vi "Test - Add Property to Schema.vi"   [LabVIEW 2020, in "JSON Schema Generator.lvlib"]
uses:
  JSON Schema Generator.lvlib
  <vilib>/addons/_JKI Toolkits/Caraya/classes/Test/Test.lvclass
  <vilib>/addons/_JKI Toolkits/Caraya/classes/Assert/Assert.lvclass
  <vilib>/JDP Science/JSONtext/JSONtext.lvlib
  <vilib>/addons/_JKI Toolkits/Caraya/classes/Assert/Assert Equal Value_Variant.vi
  <vilib>/addons/_JKI Toolkits/Caraya/classes/Assert/Assert Not Error.vi
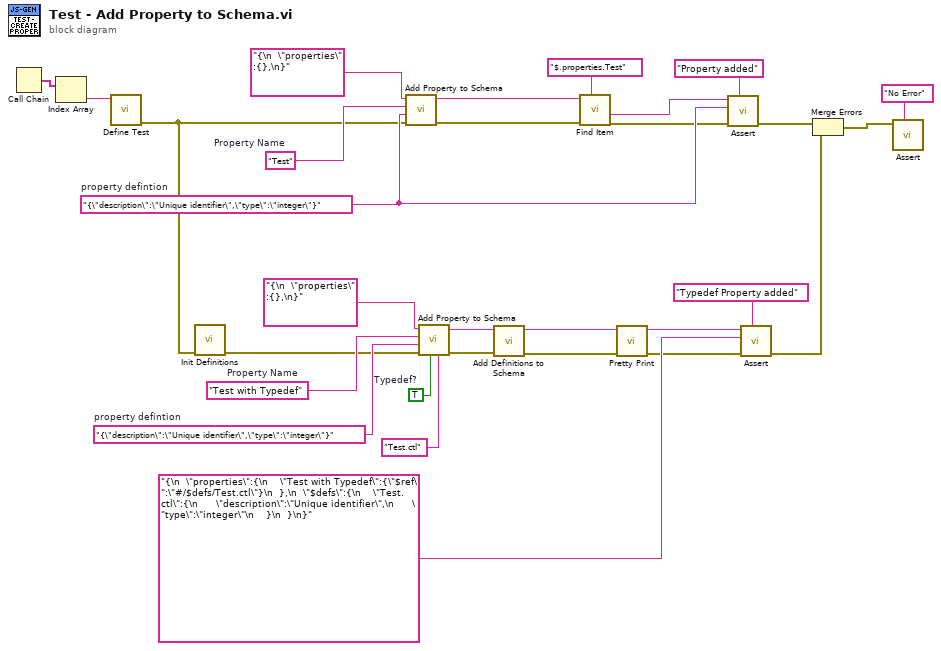
[diagram p0: block diagram]
diagram:
  w11 = TRUE  # Typedef?
  w15 = "{\"description\":\"Unique identifier\",\"type\":\"integer\"}"  # property defintion
  w17 = "Test with Typedef"  # Property Name
  w21 = "{\"description\":\"Unique identifier\",\"type\":\"integer\"}"  # property defintion
  w24 = "Test"  # Property Name
  n1 = Call Chain() -> (call chain=w30:string[])
  n2 = Index Array(array=w30) -> (element=w29:string)  [unwired: 1 in]
  n3 = call <vilib>:"Define Test.vi"("Label (VI Title)"=w29) -> ("error out"=w2:errorcluster)  [unwired: 9 in, 1 out]
  n4 = call "Init Definitions.vi"("error in (no error)"=w2) -> ("error out (no error)"=w1:errorcluster)  [unwired: 10 in]
  n5 = call "Add Property to Schema.vi"("error in"=w2, "JSON Schema Property in"=w21, "Property Name"=w24, "JSON Schema in"="{\n  \"properties\" :{},\n}") -> ("error out"=w9:errorcluster, "JSON Schema out"=w10:string)  [unwired: 6 in]
  n6 = call "Add Property to Schema.vi"("Typedef Name"="Test.ctl", "Typedef?"=w11, "error in"=w1, "JSON Schema Property in"=w15, "Property Name"=w17, "JSON Schema in"="{\n  \"properties\" :{},\n}") -> ("error out"=w7:errorcluster, "JSON Schema out"=w8:string)  [unwired: 4 in]
  n7 = call "Add Definitions to Schema.vi"("error in (no error)"=w7, "JSON In"=w8) -> ("error out"=w4:errorcluster, "JSON Out"=w6:string)  [unwired: 8 in]
  n8 = call <vilib>:"Find Item.vi"("$Path or Item Name"="$.properties.Test", "error in (no error)"=w9, "JSON"=w10) -> ("error out"=w20:errorcluster, "<JSON>"=w22:string)  [unwired: 5 in, 2 out]
  n9 = call <vilib>:"Pretty Print.vi"("error in (no error)"=w4, "JSON"=w6) -> ("error out"=w3:errorcluster, "<JSON>"=w5:string)  [unwired: 7 in, 1 out]
  n10 = call-poly <vilib>:"Assert.vi"("Label"="Property added", "error in (no error)"=w20, "Actual"=w21, "Expected"=w22) -> ("error out"=w27:errorcluster)  [unwired: 6 in, 1 out]
  n11 = call-poly <vilib>:"Assert.vi"("Label"="Typedef Property added", "error in (no error)"=w3, "Actual"="{\n  \"properties\":{\n    \"Test with Typedef\":{\"$ref\":\"#/$defs/Test.ctl\"}\n  },\n  \"$defs\":{\n    \"Test.ctl\":{\n      \"description\":\"Unique identifier\",\n      \"type\":\"integer\"\n    }\n  }\n}", "Expected"=w5) -> ("error out"=w13:errorcluster)  [unwired: 6 in, 1 out]
  n12 = Merge Errors(w27, w13) -> (w25:errorcluster)
  n13 = call-poly <vilib>:"Assert.vi"("Label"="No Error", "Not Error?"=w25) -> ()  [unwired: 8 in, 2 out]
